vi "lvmcp_staticvi.vi"() -> ()   [LabVIEW 2015]
panel:
  out "error out":errorcluster
  in  "strict":bool
  in  "path":path
  in  "reference":refnum<vi>
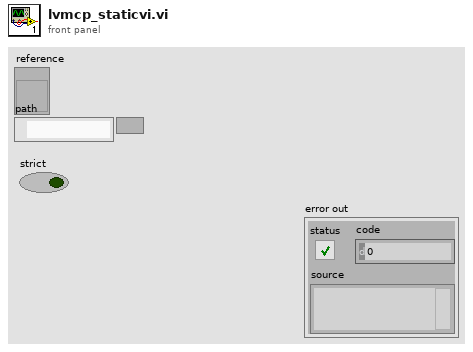
[diagram p1: front panel]
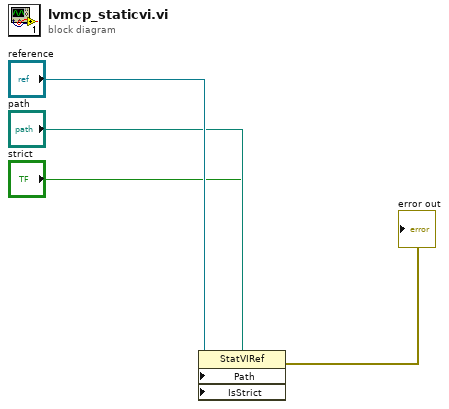
[diagram p0: block diagram]
diagram:
  n1 = property class="StatVIRef"(reference="reference", "Path"="path", "IsStrict"="strict") -> (error out=→"error out":errorcluster)  [unwired: 1 in, 1 out]
